vi "DVR Get Text Translation.vi"(8 "error in (no error)":errorcluster, 11 "Constante":string) -> (0 "error out":errorcluster, 3 "Constante":T1)   [LabVIEW 2019, in "Language Selection.lvlib"]
doc: "Converts the Data Value Reference back into Controls translation.\n- - -\nCopyright (c) 2026, Merecs Engineering GmbH"
uses:
  Language Selection.lvlib
  TypeDefs/Cluster LanguageClusterWithRefnum.ctl
  TypeDefs/Cluster PropertyTranslation.ctl
  TypeDefs/Enum Property Type.ctl
  Global Language Selection.vi
panel:
  # "Connector Pane"
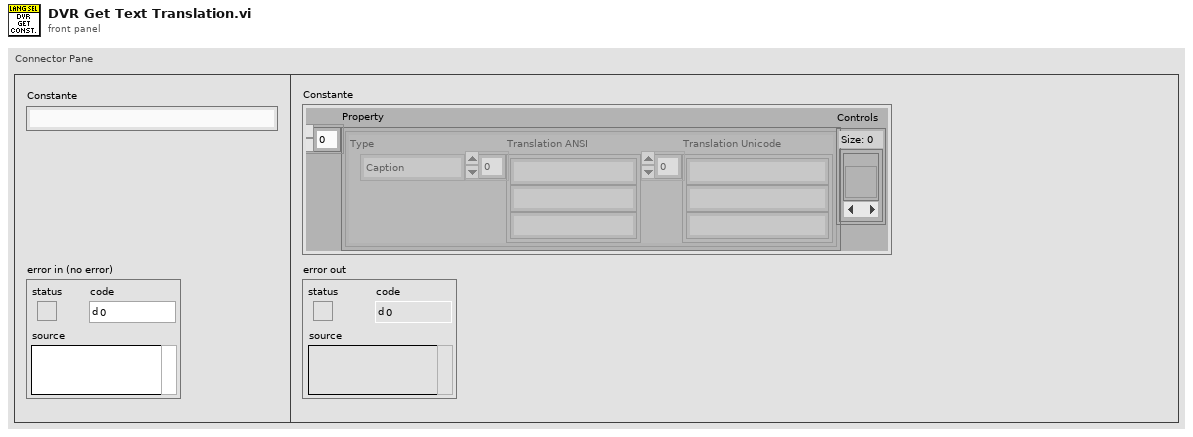
[diagram p1: front panel]
types:
  T1 = typedef "Language Selection.lvlib/Cluster LanguageClusterWithRefnum.ctl" = cluster{"Property":T2[], "Controls":set{refnum<vi>}}
  T2 = typedef "Language Selection.lvlib/Cluster PropertyTranslation.ctl" = cluster{"Type":T3, "Translation ANSI":string[], "Translation Unicode":string[]}
  T3 = typedef "Language Selection.lvlib/Enum Property Type.ctl" = enum16{"NA", "Caption", "String Value", "Boolean Text", "Ring Strings", "1D Array Elements", "2D Array Elements", "(MC)Listbox Header", "(MC)Listbox Items", "Tab Pages Names", "X & Y GraphChart", "Plot Names", "Table Headers", "Table Items", "TipStrip", "Combobox Strings", "Cursor Name", "Tree Col Headers"}
  T4 = typedef "Language Selection.lvlib/Cluster DVR.ctl" = cluster{"Data":T5, "VIs":path[], "FP Translation":map{string, T1}, "Text Translation":map{string, T1}, "Front panels":set{refnum<vi>}}
  T5 = typedef "Language Selection.lvlib/Cluster Settings Data.ctl" = cluster{"Startup Language":string, "Default Language":string, "Languages":cluster{"ANSI":string[], "Unicode":string[]}}
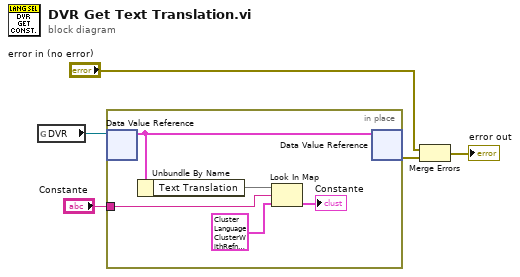
[diagram p0: block diagram]
diagram:
  n1 = global read "Global Language Selection.vi" "DVR"() -> (w5:refnum<data-value>)
  n2 = in-place {
    in-place-border: "Constante" -> [w8]
    n3 = in-place-dvr #1(w5) -> (w10:T4)  [unwired: 1 out]
    n4 = Unbundle By Name(w10) -> ("Text Translation"=w9:map{string, T1})
    n5 = Look In Map(map=w9, key=w8, default value=T1 {"Property"=[], "Controls"={}} ("f")) -> (value=→"Constante":T1)  [unwired: 1 out]
    n6 = in-place-dvr #1(w10) -> (w3:errorcluster)  [unwired: 1 out]
  }
  n7 = Merge Errors("error in (no error)", w3) -> (→"error out":errorcluster)
